vi "Write Connection.vi"(8 "error in (no error)":errorcluster, 10 "PQ Conn":refnum<class "PQ Connection.lvclass">, 11 "DBC in":refnum<class "DBC.lvclass">) -> (0 "error out":errorcluster, 3 "DBC out":refnum<class "DBC.lvclass">)   [LabVIEW 2020, in "ORM_pgsql_jdp.lvlib" / "DBC.lvclass"]
uses:
  DBC.lvclass
  <vilib>/JDP Science/PostgreSQL Library/Connection/PQ Connection.lvclass
  DBC.lvclass/DBC.ctl
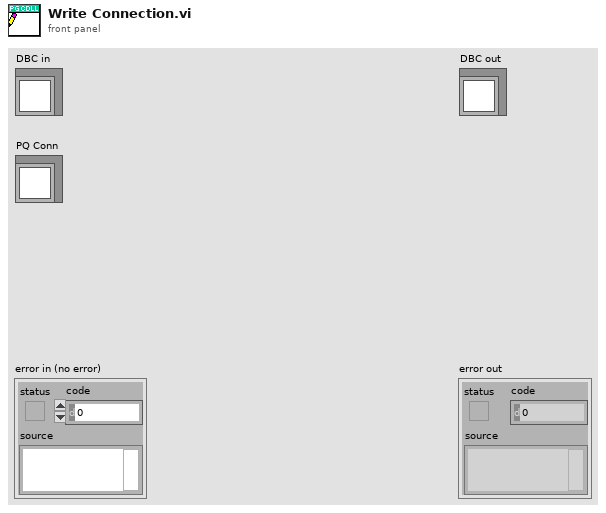
[diagram p1: front panel]
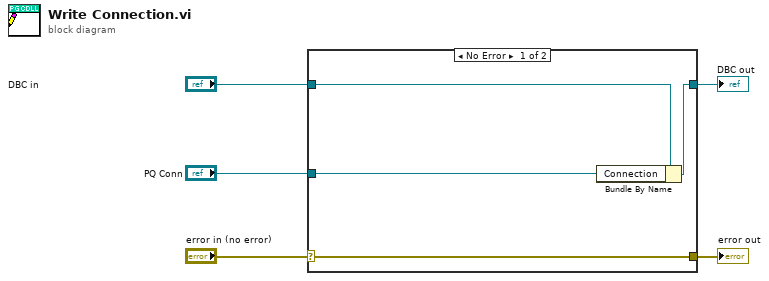
[diagram p0: block diagram]
diagram:
  n1 = case shown="No Error" "error in (no error)" {
    selector: "error in (no error)" -> [w9 w10]
    tunnel: [w9 w10] -> w4
    tunnel: [w7 w11] -> w2
    tunnel: "DBC in" -> [w8 w11]
    tunnel: "PQ Conn" -> [w6 _]
    frame No Error {
      n2 = Bundle By Name(cluster=w8, "Connection"=w6) -> (w7:refnum<class "DBC.lvclass">)
    }
    frame Error {
    }
  }
  "error out" <- w4
  "DBC out" <- w2
